vi "RemoteVI List Windows.vi"(0 "panel hWnd":u64, 5 "state":T1, 11 "error in":errorcluster) -> (4 "windows":T2(array[cluster]), 6 "modal?":bool, 8 "state out":T1, 10 "candidates":u64[](array[numeric]), 15 "error out":errorcluster)   [LabVIEW 2020, in "RemoteVI.lvlib"]
doc: "Lists the application's other windows (docs\\protocol.md section 7), front-most first. Walks the top-level windows with FindWindowExW (Z order, no callback) from the top down to the panel's owner (user32 GetWindow.vi GW_OWNER, LabVIEW's hidden frame window LVFrame, which owns the panels, LabVIEW's dialogs and the native file dialogs - an owned window is always above its owner, so the walk stops there; the whole desktop took 126 ms per call with 860 top-level windows, measured) or to the end when the panel has no owner; a CANDIDATE is a window of LabVIEW's process that is not panel hWnd, not a popup (RemoteVI Window Popup Info.vi - menus, tip strips, shadows and every captionless WS_POPUP window are popups and go to the OVERLAY instead) and has a size (LabVIEW's hidden frame window LVFrame is 0 x 0). A candidate of ANOTHER process (a window target: that process is the application, there are no IDE windows to leave out) is always LISTED - every visible, sized top-level window of it that is not the shared window and not a popup, menu, tip strip or shadow, so a non-modal window it opens (a floating inspector) is listed too. A candidate of this LabVIEW is LISTED when it is a native dialog (class #32770), when it was listed before, when it appeared while the published panel is disabled (user32 IsWindowEnabled.vi FALSE while the panel is visible - a modal dialog is up; a closed panel's stale handle is neither enabled nor visible and must not count as modal, or the server loop would never again make a VI Server call and miss the VI stopping; LabVIEW disables all its windows then and owns its own dialogs by the hidden frame window, not by the panel, measured on LabVIEW 2025), or when its owner chain (user32 GetWindow.vi GW_OWNER, up to 8 steps) reaches the panel or another such window. IDE windows that were there before (Project Explorer, block diagrams, other VIs) are not listed. APPEARED means not in the baseline: while the panel is enabled the baseline is the candidate set of the previous call, so a dialog that shows up one iteration before LabVIEW disables the panel still counts; while it is disabled the baseline is kept. The first call only takes the baseline. Each listed window is described by RemoteVI Window Info.vi (caption as JSON literal, client area in main-frame coordinates, modal, active, closable). Win32 calls only, no VI Server, so it works while a dialog or a popup holds LabVIEW's UI thread."
uses:
  RemoteVI.lvlib
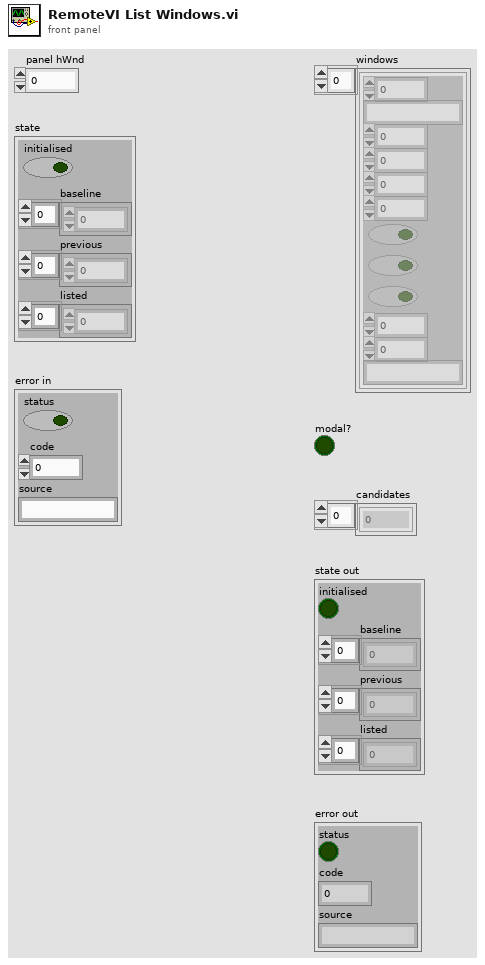
[diagram p1: front panel]
types:
  T1 = cluster{"initialised":bool, "baseline":u64[], "previous":u64[], "listed":u64[]}
  T2 = cluster{"id":u64, "title":string, "x":i32, "y":i32, "w":i32, "h":i32, "modal":bool, "active":bool, "closable":bool, "sx":i32, "sy":i32, "class":string}[]
  T3 = cluster{"hwnd":u64, "x":i32, "y":i32, "w":i32, "h":i32, "class":string}
  T4 = cluster{"id":u64, "title":string, "x":i32, "y":i32, "w":i32, "h":i32, "modal":bool, "active":bool, "closable":bool, "sx":i32, "sy":i32, "class":string}
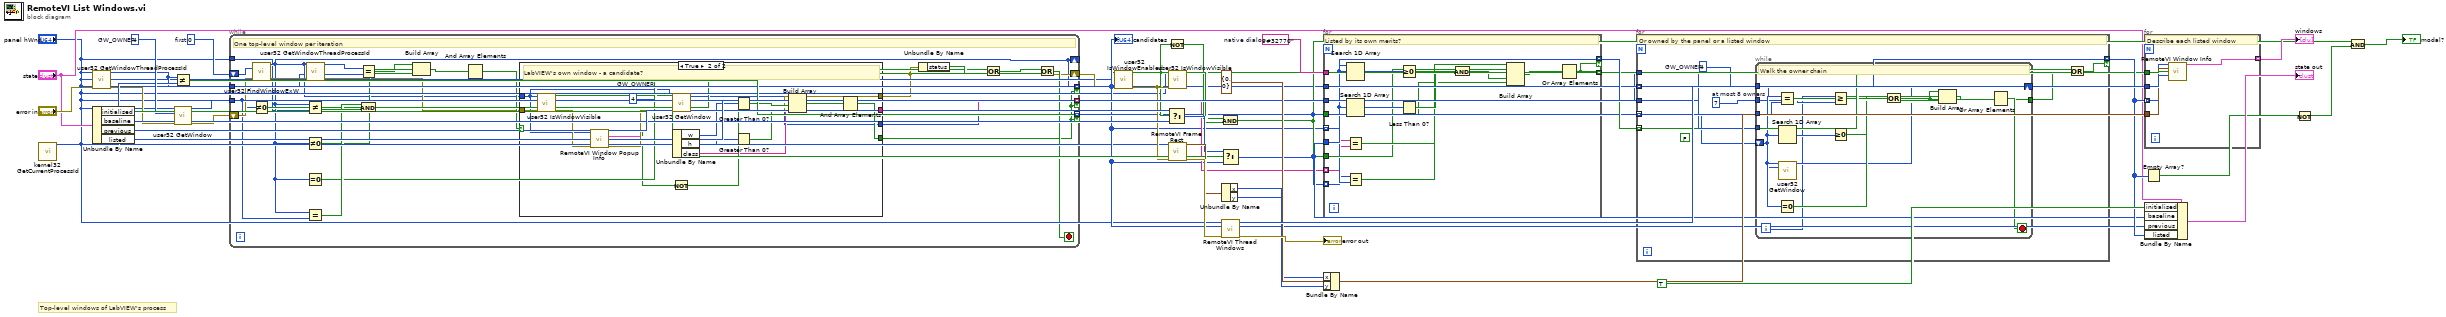
[diagram p0: block diagram]
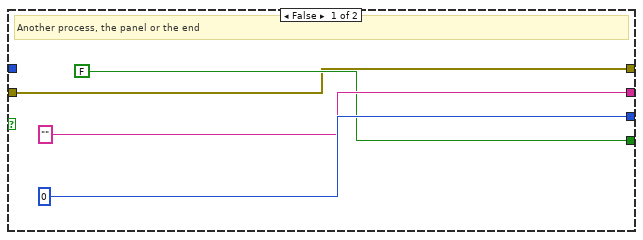
[diagram p2: hidden frame]
diagram:
  w27 = "#32770"  # native dialog
  w9 = u32 4  # GW_OWNER
  w8 = u64 0  # first
  # "Top-level windows of LabVIEW's process"
  n1 = call "kernel32 GetCurrentProcessId.vi"() -> ("process ID"=w6:u32)  [unwired: 14 in, 1 out]
  n2 = call "user32 GetWindowThreadProcessId.vi"("hWnd"="panel hWnd", "error in"="error in") -> ("process ID"=w4:u32, "error out"=w5:errorcluster)  [unwired: 11 in, 1 out]
  n3 = Unbundle By Name("state") -> ("initialised"=w21:bool, "baseline"=w22:u64[], "previous"=w23:u64[], "listed"=w24:u64[])
  n4 = Not Equal?(x=w4, y=w6) -> (x != y?=w7:bool)
  n5 = call "user32 GetWindow.vi"("hWnd"="panel hWnd", "uCmd"=w9, "error in"=w5) -> ("window"=w10:u64, "error out"=w11:errorcluster)  [unwired: 11 in]
  n6 = while {
    tunnel: "panel hWnd" -> [w46]
    shift-right: [w49] -> _
    shift-left: w8 -> [w48]
    tunnel: w4 -> [w45]
    tunnel: w10 -> [w47]
    shift-right: [w51] -> w12
    shift-left: w11 -> [w50]
    tunnel: [w49] -> w13 mode=indexing if=w60
    tunnel: [w61] -> w14 mode=indexing if=w60
    tunnel: [w62] -> w15 mode=indexing if=w60
    stop <- w69 stop-if-true
    # "One top-level window per iteration"
    n7 = call "user32 FindWindowExW.vi"("hWndChildAfter"=w48, "error in"=w50) -> ("hWnd"=w49:u64, "error out"=w52:errorcluster)  [unwired: 12 in]
    n8 = Not Equal To 0?(x=w47) -> (x != 0?=w66:bool)
    n9 = call "user32 GetWindowThreadProcessId.vi"("hWnd"=w49, "error in"=w52) -> ("process ID"=w53:u32, "error out"=w54:errorcluster)  [unwired: 11 in, 1 out]
    n10 = Not Equal?(x=w49, y=w46) -> (x != y?=w56:bool)
    n11 = Not Equal To 0?(x=w49) -> (x != 0?=w57:bool)
    n12 = Equal To 0?(x=w49) -> (x = 0?=w63:bool)
    n13 = Equal?(x=w49, y=w47) -> (x = y?=w65:bool)
    n14 = Equal?(x=w53, y=w45) -> (x = y?=w55:bool)
    n15 = And(x=w65, y=w66) -> (x .and. y?=w67:bool)
    n16 = Build Array(w55, w56, w57) -> (w58:bool[])
    n17 = And Array Elements(Boolean array=w58) -> (logical AND=w59:bool)
    n18 = case shown="True" w59 {
      tunnel: w49 -> [_ w74]
      tunnel: w54 -> [w70 w75]
      tunnel: [w70 w83] -> w51
      tunnel: ["" w86] -> w61
      tunnel: [u64 0 w82] -> w62
      tunnel: [FALSE w91] -> w60
      frame False {
        # "Another process, the panel or the end"
      }
      frame True {
        w81 = u32 4  # GW_OWNER
        # "LabVIEW's own window - a candidate?"
        n19 = call "user32 IsWindowVisible.vi"("hWnd"=w74, "error in"=w75) -> ("visible?"=w76:bool, "error out"=w77:errorcluster)  [unwired: 12 in]
        n20 = call "RemoteVI Window Popup Info.vi"("hWnd"=w74, "error in"=w77) -> ("popup?"=w78:bool, "window"=w79:T3, "error out"=w80:errorcluster)  [unwired: 11 in]
        n21 = call "user32 GetWindow.vi"("hWnd"=w74, "uCmd"=w81, "error in"=w80) -> ("window"=w82:u64, "error out"=w83:errorcluster)  [unwired: 11 in]
        n22 = Unbundle By Name(w79) -> ("w"=w84:i32, "h"=w85:i32, "class"=w86:string)
        n23 = Not(x=w78) -> (.not. x?=w87:bool)
        n24 = Greater Than 0?(x=w84) -> (x > 0?=w88:bool)
        n25 = Greater Than 0?(x=w85) -> (x > 0?=w89:bool)
        n26 = Build Array(w76, w87, w88, w89) -> (w90:bool[])
        n27 = And Array Elements(Boolean array=w90) -> (logical AND=w91:bool)
      }
    }
    n28 = Unbundle By Name(w51) -> ("status"=w64:bool)
    n29 = Or(x=w63, y=w64) -> (x .or. y?=w68:bool)
    n30 = Or(x=w68, y=w67) -> (x .or. y?=w69:bool)
  }
  "candidates" <- w13
  n31 = call "user32 IsWindowEnabled.vi"("hWnd"="panel hWnd", "error in"=w12) -> ("enabled?"=w16:bool, "error out"=w17:errorcluster)  [unwired: 12 in]
  n32 = Not(x=w16) -> (.not. x?=w18:bool)
  n33 = call "user32 IsWindowVisible.vi"("hWnd"="panel hWnd", "error in"=w17) -> ("visible?"=w19:bool)  [unwired: 12 in, 1 out]
  n34 = Select(t=w23, s=w16, f=w22) -> (s? t:f=w25:u64[])
  n35 = call "RemoteVI Frame Rect.vi"("hWnd"="panel hWnd", "error in"=w17) -> ("rect"=w31:cluster{"x":i32, "y":i32, "w":i32, "h":i32}, "error out"=w32:errorcluster)  [unwired: 12 in]
  n36 = And(x=w18, y=w19) -> (x .and. y?=w20:bool)
  n37 = Select(t=w25, s=w21, f=w13) -> (s? t:f=w26:u64[])
  n38 = Unbundle By Name(w31) -> ("x"=w33:i32, "y"=w34:i32)
  n39 = call "RemoteVI Thread Windows.vi"("hWnd"="panel hWnd", "error in"=w32) -> ("active"=w37:u64, "error out"=→"error out":errorcluster)  [unwired: 10 in, 2 out]
  n40 = for {
    tunnel: w27 -> [w95]
    tunnel: "panel hWnd" -> [w96]
    tunnel: w24 -> [w97]
    tunnel: w7 -> [w100]
    tunnel: w13 -> [w92] mode=indexing
    tunnel: w26 -> [w98]
    tunnel: w20 -> [w99]
    tunnel: [w92] -> w29 mode=indexing if=w109
    tunnel: w14 -> [w93] mode=indexing
    tunnel: w15 -> [w94] mode=indexing
    tunnel: [w109] -> w28 mode=indexing
    # "Listed by its own merits?"
    n41 = Search 1D Array(1D array=w97, element=w92) -> (index of element=w103:i32)  [unwired: 1 in]
    n42 = Search 1D Array(1D array=w98, element=w92) -> (index of element=w105:i32)  [unwired: 1 in]
    n43 = Equal?(x=w93, y=w95) -> (x = y?=w101:bool)
    n44 = Equal?(x=w94, y=w96) -> (x = y?=w102:bool)
    n45 = Greater Or Equal To 0?(x=w103) -> (x >= 0?=w104:bool)
    n46 = Less Than 0?(x=w105) -> (x < 0?=w106:bool)
    n47 = And(x=w99, y=w106) -> (x .and. y?=w107:bool)
    n48 = Build Array(w101, w102, w104, w107, w100) -> (w108:bool[])
    n49 = Or Array Elements(Boolean array=w108) -> (logical OR=w109:bool)
  }
  n50 = Bundle By Name(cluster=cluster{"x":i32, "y":i32} {"x"=0, "y"=0}, "x"=w33, "y"=w34) -> (w36:cluster{"x":i32, "y":i32})
  n51 = for {
    tunnel: "panel hWnd" -> [w114]
    tunnel: w13 -> [w110] mode=indexing
    tunnel: [w110] -> w30 mode=indexing if=w118
    tunnel: w29 -> [w113]
    tunnel: w15 -> [w111] mode=indexing
    tunnel: w28 -> [w112] mode=indexing
    (unwired) FALSE
    w116 = 7  # at most 8 owners
    w115 = u32 4  # GW_OWNER
    # "Or owned by the panel or a listed window"
    n52 = while {
      tunnel: w115 -> [w122]
      tunnel: w116 -> [w123]
      tunnel: w114 -> [w121]
      tunnel: w113 -> [w120]
      shift-right: [w125] -> _
      shift-left: w111 -> [w124]
      tunnel: [w129] -> w117
      i -> [w119]
      stop <- w133 stop-if-true
      # "Walk the owner chain"
      n53 = Equal?(x=w124, y=w121) -> (x = y?=w126:bool)
      n54 = Search 1D Array(1D array=w120, element=w124) -> (index of element=w127:i32)  [unwired: 1 in]
      n55 = call "user32 GetWindow.vi"("hWnd"=w124, "uCmd"=w122) -> ("window"=w125:u64)  [unwired: 12 in, 1 out]
      n56 = Equal To 0?(x=w124) -> (x = 0?=w130:bool)
      n57 = Greater Or Equal?(x=w119, y=w123) -> (x >= y?=w131:bool)
      n58 = Greater Or Equal To 0?(x=w127) -> (x >= 0?=w128:bool)
      n59 = Or(x=w126, y=w128) -> (x .or. y?=w129:bool)
      n60 = Build Array(w129, w130, w131) -> (w132:bool[])
      n61 = Or Array Elements(Boolean array=w132) -> (logical OR=w133:bool)
    }
    n62 = Or(x=w112, y=w117) -> (x .or. y?=w118:bool)
  }
  n63 = for {
    tunnel: w16 -> [w136]
    tunnel: w37 -> [w137]
    tunnel: w30 -> [w134] mode=indexing
    tunnel: w36 -> [w135]
    tunnel: [w138] -> w39 mode=indexing
    # "Describe each listed window"
    n64 = call "RemoteVI Window Info.vi"("hWnd"=w134, "frame origin"=w135, "panel enabled?"=w136, "active"=w137) -> ("window"=w138:T4)  [unwired: 10 in, 1 out]
  }
  "windows" <- w39
  n65 = Empty Array?(array=w30) -> (empty?=w40:bool)
  n66 = Bundle By Name(cluster="state", "initialised"=TRUE, "baseline"=w26, "previous"=w13, "listed"=w30) -> (→"state out":T1)
  n67 = Not(x=w40) -> (.not. x?=w41:bool)
  n68 = And(x=w20, y=w41) -> (x .and. y?=→"modal?":bool)
